vi "ZM-CP-publish.vi"(8 "error in (no error)":errorcluster, 10 "package":refnum<class "ZM-PC-package.lvclass">, 11 "ZM-CP-MX-multi_protocol in":refnum<class "ZM-CP-MX-multi_protocol.lvclass">) -> (0 "error out":errorcluster, 3 "ZM-CP-MX-multi_protocol out":refnum<class "ZM-CP-MX-multi_protocol.lvclass">)   [LabVIEW 2020, in "ZM-CP-MX-multi_protocol.lvlib" / "ZM-CP-MX-multi_protocol.lvclass"]
doc: "The multi protocol's ZM-CP-publish: publishes the same package to every protocol in the array in order and stops at the first error, which is returned. The protocol never looks inside the package. No Call Parent."
uses:
  ZM-CP-MX-multi_protocol.lvclass
  common/ZM-PC-packages/ZM-PC-package/ZM-PC-package.lvclass
  ZM-CP-MX-multi_protocol.lvclass/ZM-CP-MX-multi_protocol.ctl
  ZM-CP-communication_protocol/ZM-CP-communication_protocol/ZM-CP-communication_protocol.lvclass
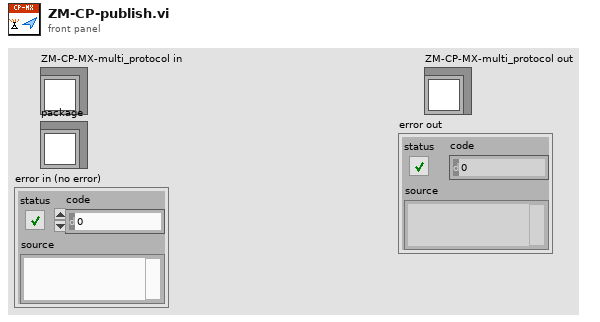
[diagram p1: front panel]
types:
  T1 = typedef "ZM-CP-MX-multi_protocol.lvlib/ZM-CP-MX-multi_protocol.lvclass/ZM-CP-MX-PROTOCOLS.ctl" = refnum<class "ZM-CP-communication_protocol.lvclass">[]
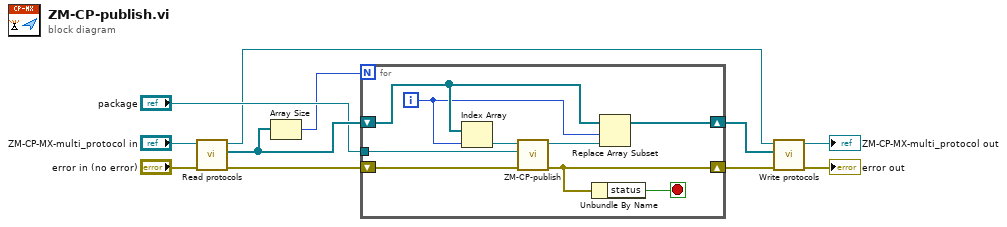
[diagram p0: block diagram]
diagram:
  n1 = call "Read protocols.vi"("error in (no error)"="error in (no error)", "ZM-CP-MX-multi_protocol in"="ZM-CP-MX-multi_protocol in") -> ("error out"=w8:errorcluster, "ZM-CP-MX-PROTOCOLS"=w9:T1, "ZM-CP-MX-multi_protocol out"=w5:refnum<class "ZM-CP-MX-multi_protocol.lvclass">)  [unwired: 7 in]
  n2 = Array Size(array=w9) -> (size(s)=w6:i32)
  n3 = for {
    N: w6 -> [_]
    shift-right: [w15] -> w4
    shift-left: w9 -> [w17]
    shift-right: [w14] -> w3
    shift-left: w8 -> [w18]
    tunnel: "package" -> [w19]
    i -> [w12]
    stop <- w13 stop-if-true
    n4 = Index Array(array=w17, index=w12) -> (element=w20:refnum<class "ZM-CP-communication_protocol.lvclass">)
    n5 = call-dynamic "ZM-CP-publish.vi"("error in (no error)"=w18, "package"=w19, "ZM-CP-communication_protocol in"=w20) -> ("error out"=w14:errorcluster, "ZM-CP-communication_protocol out"=w16:refnum<class "ZM-CP-communication_protocol.lvclass">)  [unwired: 7 in]
    n6 = Unbundle By Name(w14) -> ("status"=w13:bool)
    n7 = Replace Array Subset(array=w17, new element=w16, index=w12) -> (w15:T1)
  }
  n8 = call "Write protocols.vi"("error in (no error)"=w3, "ZM-CP-MX-PROTOCOLS"=w4, "ZM-CP-MX-multi_protocol in"=w5) -> ("error out"=→"error out":errorcluster, "ZM-CP-MX-multi_protocol out"=→"ZM-CP-MX-multi_protocol out":refnum<class "ZM-CP-MX-multi_protocol.lvclass">)  [unwired: 7 in]
